vi "Connect.vi"(8 "error in (no error)":errorcluster, 10 "Connection String":string, 11 "SqliteConnection in":refnum<class "DBC.lvclass">) -> (0 "error out":errorcluster, 3 "SqliteConnection out":refnum<class "DBC.lvclass">)   [LabVIEW 2026, in "ORM_DBC_Sqlite_netCore.lvlib" / "DBC.lvclass"]
uses:
  DBC.lvclass
  DBC.lvclass/DBC.ctl
  <vilib>/Viviota/shared/data_nc/SQLitePCLRaw.batteries_v2.dll
  <vilib>/Viviota/shared/ORM_DBC_dotNetCore.lvlibp/Write connection.vi
  <vilib>/Viviota/shared/ORM.lvlibp/DbConnection/Write ColumnNameEqualsValueFormat.vi
  <vilib>/Viviota/shared/ORM.lvlibp/DbConnection/Write ColumnNameFormat.vi
  <vilib>/Viviota/shared/ORM.lvlibp/DbConnection/Write LastIdentityQuery.vi
  <vilib>/Viviota/shared/ORM.lvlibp/DbConnection/Write TableNameFormat.vi
  <vilib>/Viviota/shared/data_nc/Microsoft.Data.Sqlite.dll
  <vilib>/regexp/Match Regular Expression.xnode
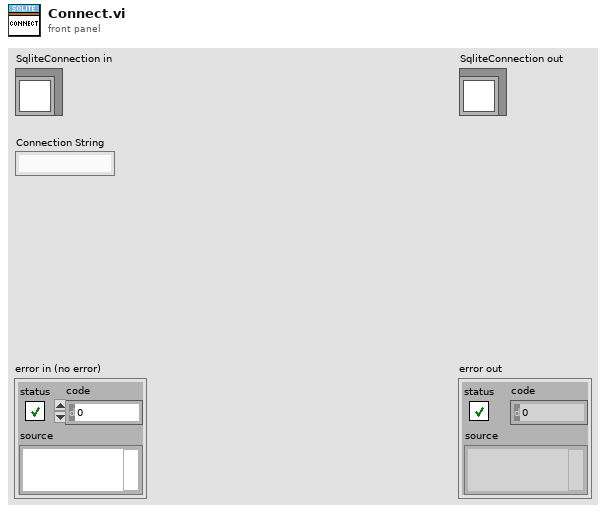
[diagram p1: front panel]
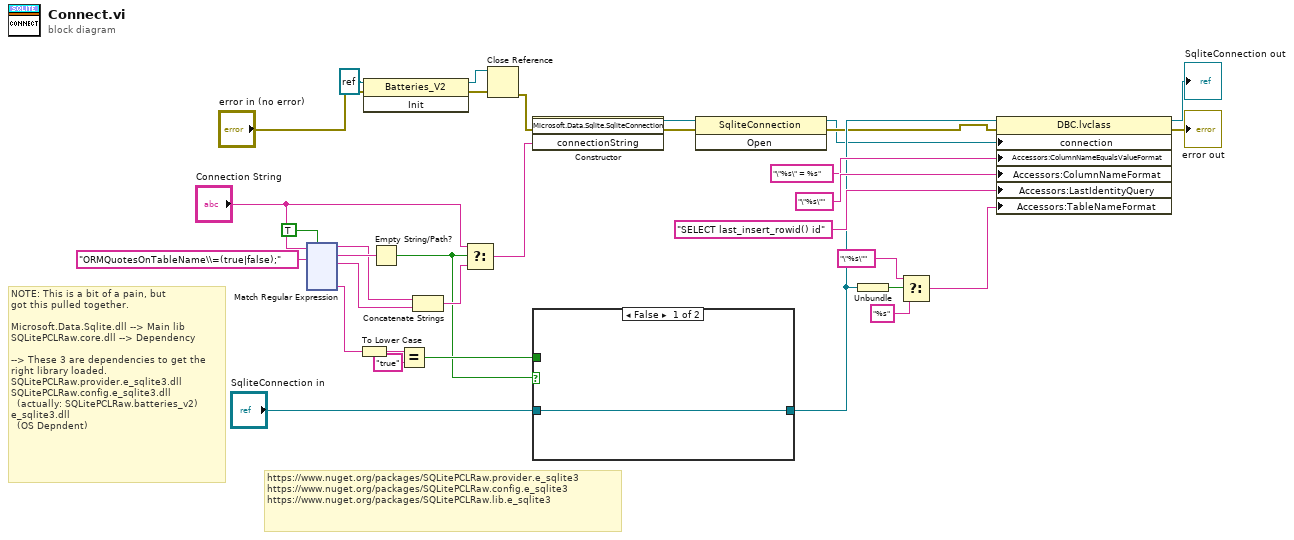
[diagram p0: block diagram]
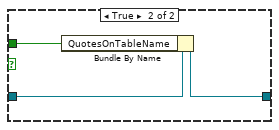
[diagram p2: hidden frame]
diagram:
  # "https://www.nuget.org/packages/SQLitePCLRaw.provider.e_sqlite3\nhttps://www.nuget.org/packages/SQLitePCLRaw.config.e_sqlite3\nhttps://www.nuget.org/packages/SQLitePCLRaw.lib.e_sqlite3"
  # "NOTE: This is a bit of a pain, but\ngot this pulled together.  \n\nMicrosoft.Data.Sqlite.dll --> Main lib\nSQLitePCLRaw.core.dll --> Dependency\n\n--> These 3 are dependencies to get the \nright library loaded.\nSQLitePCLRaw.provider.e_sqlite3.dll\nSQLitePCLRaw.config.e_sqlite3.dll\n  (actually: SQLitePCLRaw.batteries_v2)\ne_sqlite3.dll\n  (OS Depndent)"
  n1 = xnode "Match Regular Expression"("input string"="Connection String", "regular expression"="ORMQuotesOnTableName\\=(true|false);", "ignore case? (F)"=TRUE) -> ("before match"=w20:string, "whole match"=w21:string, "after match"=w19:string, "submatch 1"=w16:string)  [unwired: 3 in, 2 out]
  n2 = To Lower Case(string=w16) -> (all lower case string=w15:string)
  n3 = invoke class="Batteries_V2" method="Init"(reference=refnum<k39> refnum ("new reference"), error in="error in (no error)") -> (reference out=w3:refnum<k39>, error out=w4:errorcluster)  [unwired: 1 in, 1 out]
  n4 = Empty String/Path?(string/path=w21) -> (empty?=w11:bool)
  n5 = Equal?(x=w15, y="true") -> (x = y?=w12:bool)
  n6 = Concatenate Strings(w20, w19) -> (w17:string)
  n7 = Select(t="Connection String", s=w11, f=w17) -> (s? t:f=w9:string)
  n8 = Close Reference(reference=w3, error in (no error)=w4) -> (error out=w1:errorcluster)
  n9 = constructor class="SqliteConnection"(error in=w1, "connectionString"=w9) -> (reference out=w7:refnum<k39>, error out=w10:errorcluster)  [unwired: 2 in, 2 out]
  n10 = case shown="False" w11 {
    tunnel: "SqliteConnection in" -> [w34 w37]
    tunnel: [w34 w36] -> w13
    tunnel: w12 -> [_ w35]
    frame False {
    }
    frame True {
      n11 = Bundle By Name(cluster=w37, "QuotesOnTableName"=w35) -> (w36:refnum<class "DBC.lvclass">)
    }
  }
  n12 = invoke class="SqliteConnection" method="Open"(reference=w7, error in=w10) -> (reference out=w6:refnum<k39>, error out=w8:errorcluster)  [unwired: 1 in, 1 out]
  n13 = Unbundle(w13) -> (w27:bool)
  n14 = Select(t="\"%s\"" ("TableNameFormat"), s=w27, f="%s" ("TableNameFormat")) -> (s? t:f=w24:string)
  n15 = property class="DBC.lvclass"(reference=w13, error in=w8, "connection"=w6, "Accessors:ColumnNameEqualsValueFormat"="\"%s\" = %s" ("ColumnNameFormat"), "Accessors:ColumnNameFormat"="\"%s\"" ("ColumnNameFormat"), "Accessors:LastIdentityQuery"="SELECT last_insert_rowid() id" ("LastIdentityQuery"), "Accessors:TableNameFormat"=w24) -> (reference out=→"SqliteConnection out":refnum<class "DBC.lvclass">, error out=→"error out":errorcluster)
